vi "fake tool added later.vi"(8 "error in":errorcluster, 11 "text":string) -> (0 "error out":errorcluster, 3 "echo":string)   [LabVIEW 2020, in "MCP Server tests.lvlib"]
doc: "Test fixture: a tool that is not registered when the test server starts. Test 75 adds it to the running server and expects the next tools/list to contain it. Returns text unchanged."
uses:
  MCP Server tests.lvlib
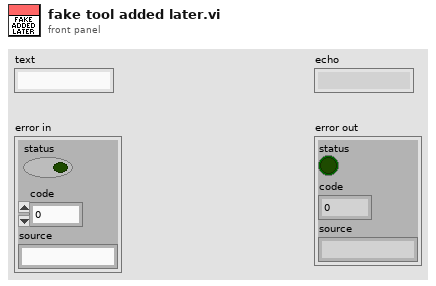
[diagram p1: front panel]
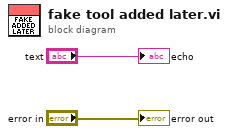
[diagram p0: block diagram]
diagram:
  "echo" <- "text"
  "error out" <- "error in"
